vi "SPARK Set Output.vi"(4 "Arbitrary Feed Forward (0)":dbl, 6 "Closed Loop Slot":T3 items=["Slot 0", "Slot 1", "Slot 2", "Slot 3"], 8 "error in (no error)":errorcluster, 9 "Control Mode":T2, 10 "Setpoint":dbl(slide) scale=-1.0..1.0, 11 "Spark refnum":T1) -> (0 "error out":errorcluster, 3 "Spark refnum":T1)   [LabVIEW 2023, in "REVLibDriver.lvlib"]
uses:
  <vilib>/REVLibDriver/REVLibDriver.lvlib
  <vilib>/REV Custom Controls/SPARK Closed Loop Slot.ctl
  <vilib>/REV Custom Controls/Spark Output Control Type.ctl
  <vilib>/REV Custom Controls/REVSparkRefnum.ctl
  <vilib>/REV Custom Controls/c_Spark_ControlType.ctl
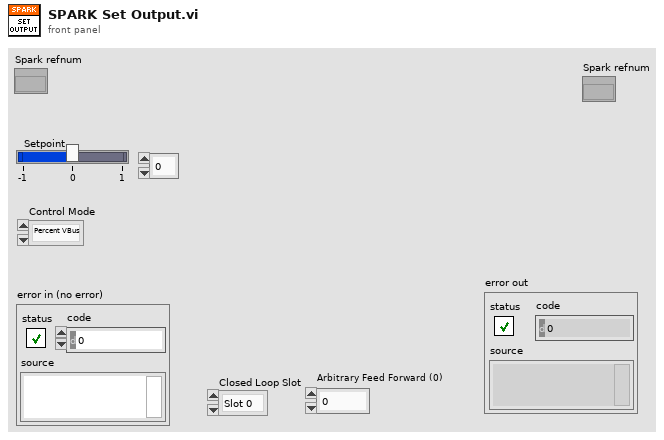
[diagram p1: front panel]
types:
  T1 = typedef "REVLibDriver.lvlib/REVSparkRefnum.ctl" = refnum<k20>
  T2 = typedef "REVLibDriver.lvlib/Spark Output Control Type.ctl" = enum16{"Percent VBus", "Velocity", "Voltage", "Position", "Current", "MAXMotion Position", "MAXMotion Velocity"}
  T3 = typedef "SPARK Closed Loop Slot.ctl" = u16
  T4 = typedef "REVLibDriver.lvlib/c_Spark_ControlType.ctl" = enum16{"c_Spark_kControlType_DUTY_CYCLE", "    c_Spark_kControlType_VELOCITY", "    c_Spark_kControlType_VOLTAGE", "    c_Spark_kControlType_POSITION", "    c_Spark_kControlType_CURRENT", "    c_Spark_kControlType_MAXMOTION_POSITION", "    c_Spark_kControlType_MAXMOTION_VELOCITY", "    c_Spark_kNumControlTypes"}
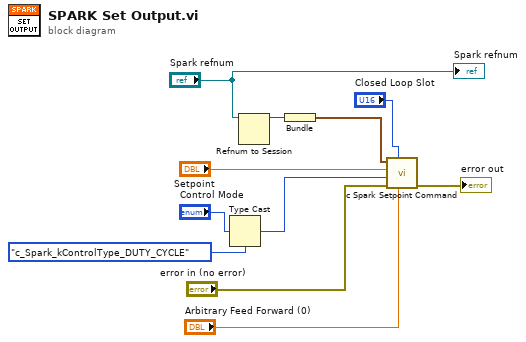
[diagram p0: block diagram]
diagram:
  n1 = Type Cast(type=c_Spark_ControlType."c_Spark_kControlType_DUTY_CYCLE" ("ctrl"), x="Control Mode") -> (*(type *) &x=w4:T4)
  n2 = Refnum to Session(7:"Spark refnum") -> (3:w3:u64)  [unwired: 1 in, 1 out]
  n3 = Bundle("Session"=w3) -> (w2:cluster{"Session":u64})  [unwired: 1 in]
  n4 = call <vilib>:"c Spark Setpoint Command.vi"("arbFeedforward"="Arbitrary Feed Forward (0)", "pidSlot"="Closed Loop Slot", "error in (no error)"="error in (no error)", "ctrl"=w4, "value"="Setpoint", "handle"=w2) -> ("error out"=→"error out":errorcluster)  [unwired: 3 in, 2 out]
  "Spark refnum" <- "Spark refnum"
